vi "set Modulation.vi"(8 "error in (no error)":errorcluster, 10 "Modulation":T1, 11 "LTE in":refnum<class "LTE.lvclass">) -> (0 "error out":errorcluster, 3 "LTE out":refnum<class "LTE.lvclass">)   [LabVIEW 2023, in "ANRITSU Call Box.lvlib" / "LTE.lvclass"]
uses:
  LTE.lvclass
  LTE.lvclass/LTE.ctl
  Type Definition/LTE Modulation Type.ctl
  ANRITSU Call Box.lvlib
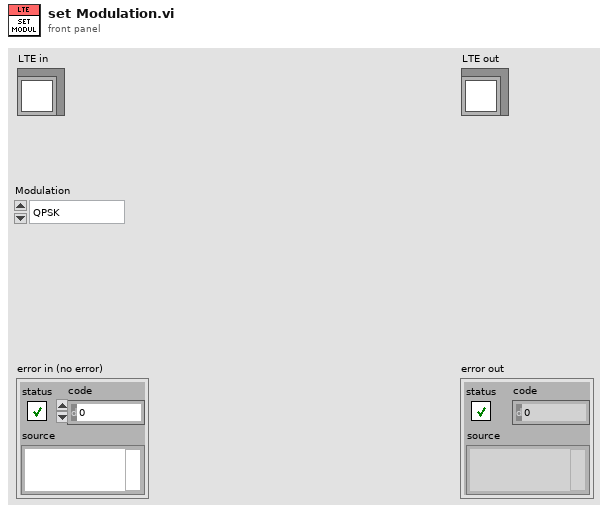
[diagram p1: front panel]
types:
  T1 = typedef "ANRITSU Call Box.lvlib/LTE Modulation Type.ctl" = enum16{"QPSK", "16QAM", "64QAM", "256QAM"}
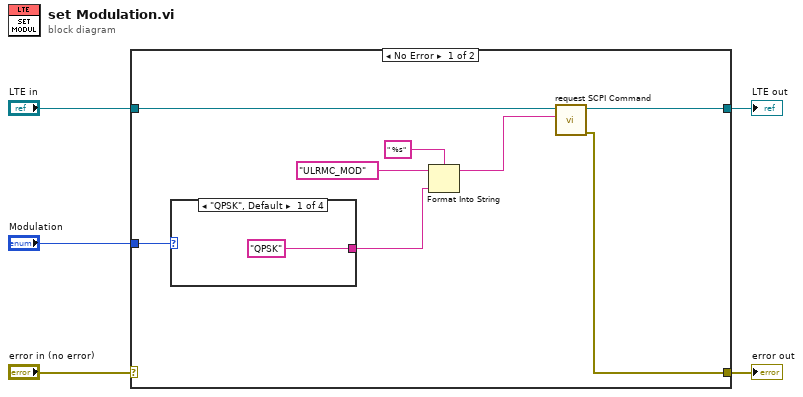
[diagram p0: block diagram]
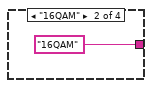
[diagram p2: hidden frame]
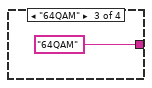
[diagram p3: hidden frame]
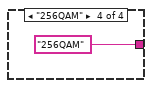
[diagram p4: hidden frame]
diagram:
  n1 = case shown="No Error" "error in (no error)" {
    selector: "error in (no error)" -> [_ w19]
    tunnel: [w6 w19] -> w4
    tunnel: [w12 w18] -> w2
    tunnel: "LTE in" -> [w13 w18]
    tunnel: "Modulation" -> [w11 _]
    frame No Error {
      n2 = case shown="\"QPSK\", Default" w11 {
        tunnel: ["QPSK" "16QAM" "64QAM" "256QAM"] -> w8
        frame "QPSK", Default {
        }
        frame "16QAM" {
        }
        frame "64QAM" {
        }
        frame "256QAM" {
        }
      }
      n3 = Format Into String(format string=" %s", initial string="ULRMC_MOD", w8) -> (resulting string=w7:string)  [unwired: 1 in, 1 out]
      n4 = call "request SCPI Command.vi"("SCPI Command"=w7, "LTE in"=w13) -> ("error out"=w6:errorcluster, "LTE out"=w12:refnum<class "LTE.lvclass">)  [unwired: 8 in]
    }
    frame Error {
    }
  }
  "error out" <- w4
  "LTE out" <- w2
